vi "Close.vi"(8 "error in (no error)":errorcluster, 11 "Motor in":refnum<class "Motor.lvclass">) -> (0 "error out":errorcluster, 3 "Motor out":refnum<class "Motor.lvclass">)   [LabVIEW 2021, in "Motor.lvclass"]
doc: "This VI forces servodrive command to 0V and disable servodrive. Finally close all references."
uses:
  Motor.lvclass
  Motor.lvclass/Motor.ctl
  AnalogInput/AnalogInput.lvclass
  AnalogOutput/AnalogOutput.lvclass
  ServoDrive/ServoDrive.lvclass
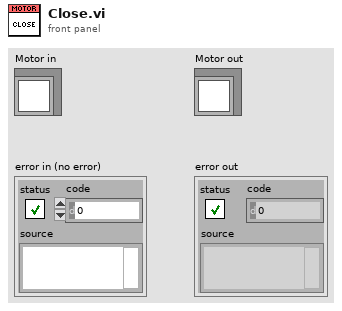
[diagram p1: front panel]
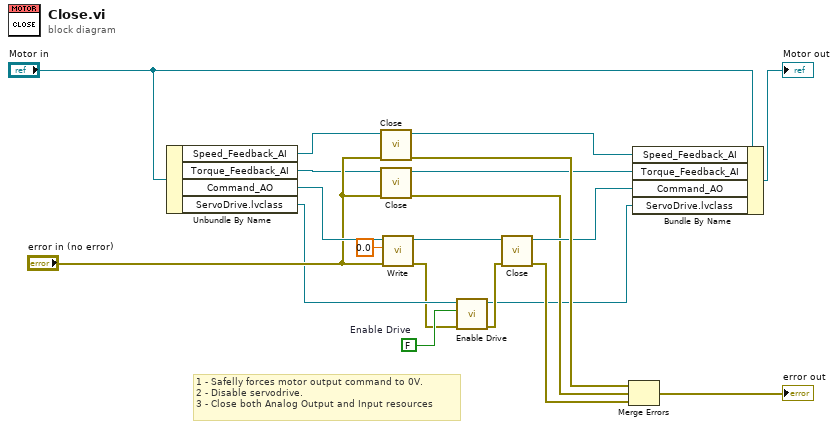
[diagram p0: block diagram]
diagram:
  w5 = FALSE  # Enable Drive
  # "1 - Safelly forces motor output command to 0V.\n2 - Disable servodrive.\n3 - Close both Analog Output and Input resources"
  n1 = Unbundle By Name("Motor in") -> ("Speed_Feedback_AI"=w19:refnum<class "AnalogInput.lvclass">, "Torque_Feedback_AI"=w8:refnum<class "AnalogInput.lvclass">, "Command_AO"=w10:refnum<class "AnalogOutput.lvclass">, "ServoDrive.lvclass"=w4:refnum<class "ServoDrive.lvclass">)
  n2 = call-dynamic "Close.vi"("error in (no error)"="error in (no error)", "AnalogInput in"=w19) -> ("error out"=w17:errorcluster, "AnalogInput out"=w16:refnum<class "AnalogInput.lvclass">)  [unwired: 8 in]
  n3 = call-dynamic "Close.vi"("error in (no error)"="error in (no error)", "AnalogInput in"=w8) -> ("error out"=w6:errorcluster, "AnalogInput out"=w7:refnum<class "AnalogInput.lvclass">)  [unwired: 8 in]
  n4 = call-dynamic "Write.vi"("error in (no error)"="error in (no error)", "data in"=0.0, "AnalogOutput in"=w10) -> ("error out"=w3:errorcluster, "AnalogOutput out"=w12:refnum<class "AnalogOutput.lvclass">)  [unwired: 7 in]
  n5 = call-dynamic "Enable Drive.vi"("error in (no error)"=w3, "Enable Drive"=w5, "ServoDrive in"=w4) -> ("error out"=w2:errorcluster, "ServoDrive out"=w1:refnum<class "ServoDrive.lvclass">)  [unwired: 7 in]
  n6 = call-dynamic "Close.vi"("error in (no error)"=w2, "AnalogOutput in"=w12) -> ("error out"=w18:errorcluster, "AnalogOutput out"=w13:refnum<class "AnalogOutput.lvclass">)  [unwired: 8 in]
  n7 = Merge Errors(w17, w6, w18) -> (→"error out":errorcluster)
  n8 = Bundle By Name(cluster="Motor in", "Speed_Feedback_AI"=w16, "Torque_Feedback_AI"=w7, "Command_AO"=w13, "ServoDrive.lvclass"=w1) -> (→"Motor out":refnum<class "Motor.lvclass">)
